vi "Load Class From Config.vi"(8 "error in (no error)":errorcluster, 11 "Name":string) -> (0 "error out":errorcluster, 2 "Success":bool, 3 "Channel":refnum<class "Channel.lvclass">)   [LabVIEW 2021, in "Channel.lvlib"]
doc: "Loads the class from the configuration Folder"
uses:
  Channel.lvlib
  Channel/Channel_class/Channel.lvclass
  <vilib>/Utility/config.llb/Read Key (String).vi
  <vilib>/Utility/config.llb/NI_LVConfig.lvlib
panel:
  in  "PluginPath(T)":bool=TRUE
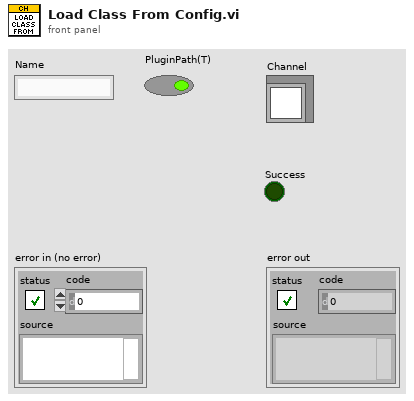
[diagram p1: front panel]
types:
  T1 = typedef "NI_LVConfig.lvlib/Config Data RefNum.ctl" = refnum<k1>
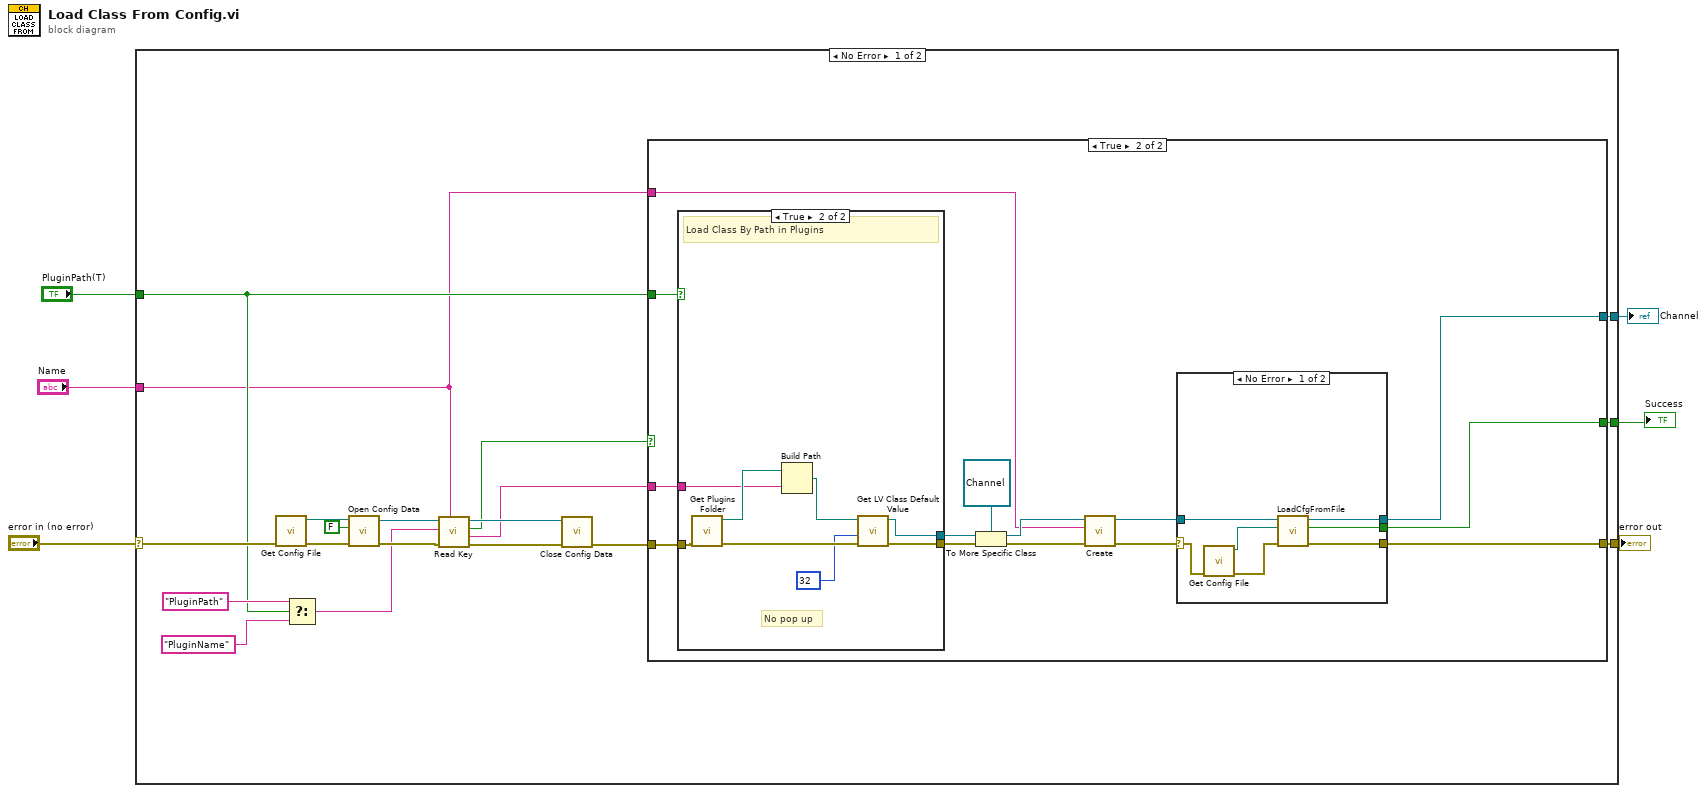
[diagram p0: block diagram]
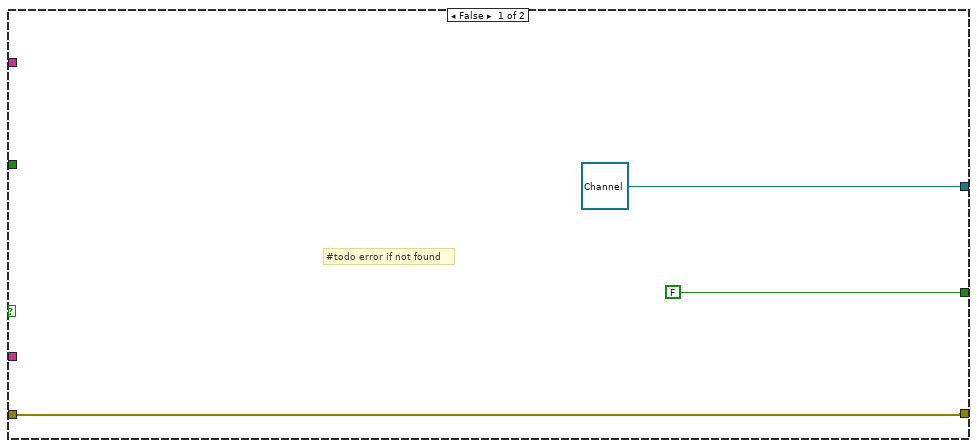
[diagram p2: hidden frame]
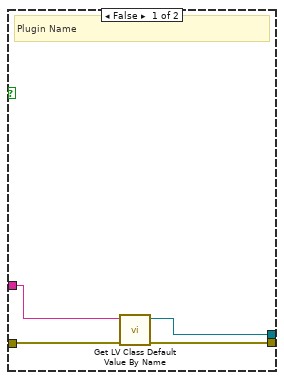
[diagram p3: hidden frame]
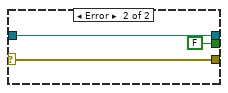
[diagram p4: hidden frame]
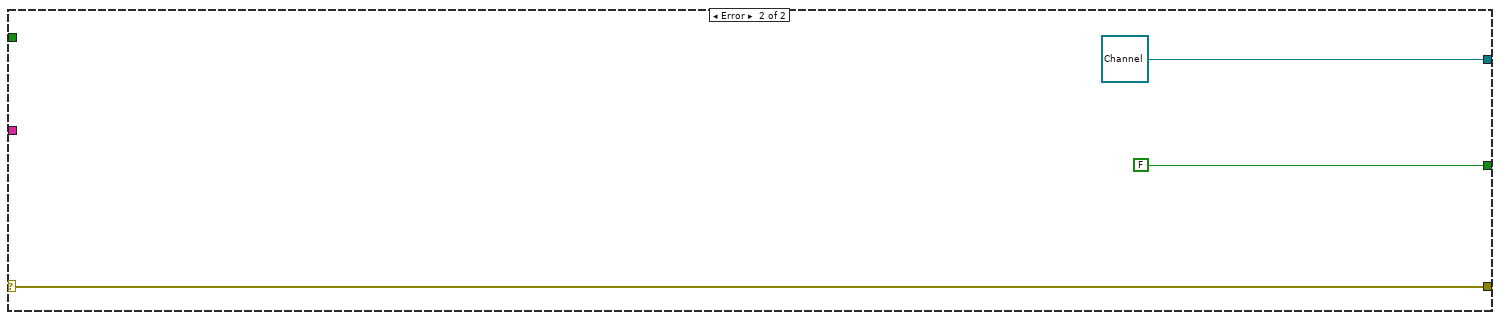
[diagram p5: hidden frame]
diagram:
  n1 = case shown="No Error" "error in (no error)" {
    selector: "error in (no error)" -> [w25 w66]
    tunnel: [w24 w66] -> w5
    tunnel: "Name" -> [w7 _]
    tunnel: [w12 FALSE ("Boolean")] -> w3
    tunnel: [w11 refnum<class "Channel.lvclass"> refnum ("Channel.lvlib:Channel")] -> w2
    tunnel: "PluginPath(T)" -> [w9 _]
    frame No Error {
      n2 = call "Get Config File.vi"("error in (no error)"=w25) -> ("error out"=w18:errorcluster, "Config File"=w21:path)  [unwired: 9 in]
      n3 = Select(t="PluginPath" ("key"), s=w9, f="PluginName") -> (s? t:f=w10:string)
      n4 = call <vilib>:"Open Config Data.vi"("error in (no error)"=w18, "create file if necessary (T)"=FALSE, "configuration file path"=w21) -> ("error out"=w19:errorcluster, "refnum"=w22:T1)  [unwired: 6 in, 1 out]
      n5 = call-poly <vilib>:"Read Key.vi"("section"=w7, "error in (no error)"=w19, "key"=w10, "refnum"=w22) -> ("error out"=w16:errorcluster, "value"=w14:string, "found?"=w13:bool, "refnum out"=w23:T1)  [unwired: 4 in]
      n6 = call <vilib>:"Close Config Data.vi"("error in (no error)"=w16, "refnum"=w23) -> ("error out"=w17:errorcluster)  [unwired: 8 in, 1 out]
      n7 = case shown="True" w13 {
        tunnel: [w28 w36] -> w24
        tunnel: w17 -> [w28 w42]
        tunnel: w14 -> [_ w41]
        tunnel: [FALSE ("Boolean") w35] -> w12
        tunnel: [refnum<class "Channel.lvclass"> refnum ("Channel.lvlib:Channel") w37] -> w11
        tunnel: w9 -> [_ w34]
        tunnel: w7 -> [_ w29]
        frame False {
          # "#todo error if not found"
        }
        frame True {
          n8 = case shown="True" w34 {
            tunnel: w42 -> [w45 w54]
            tunnel: w41 -> [w46 w52]
            tunnel: [w43 w49] -> w39
            tunnel: [w44 w48] -> w38
            frame False {
              # "Plugin Name"
              n9 = call <vilib>:"Get LV Class Default Value By Name.vi"("error in (no error)"=w45, "class name"=w46) -> ("error out"=w44:errorcluster, "object"=w43:refnum<class>)  [unwired: 8 in]
            }
            frame True {
              # "No pop up"
              # "Load Class By Path in Plugins"
              n10 = call "Get Plugins Folder.vi"("error in (no error)"=w54) -> ("error out"=w50:errorcluster, "Plugins Folder"=w53:path)  [unwired: 9 in]
              n11 = Build Path(base path=w53, name or relative path=w52) -> (appended path=w51:path)
              n12 = call <vilib>:"Get LV Class Default Value.vi"("error in (no error)"=w50, "options"=u32 32, "class path"=w51) -> ("error out"=w48:errorcluster, "object"=w49:refnum<class>)  [unwired: 7 in]
            }
          }
          n13 = To More Specific Class(target class=refnum<class "Channel.lvclass"> refnum ("Channel.lvlib:Channel"), reference=w39, error in=w38) -> (specific class reference=w33:refnum<class "Channel.lvclass">, error out=w32:errorcluster)
          n14 = call-dynamic "Create.vi"("error in (no error)"=w32, "Name"=w29, "object in"=w33) -> ("error out"=w31:errorcluster, "object out"=w30:refnum<class "Channel.lvclass">)  [unwired: 7 in]
          n15 = case shown="No Error" w31 {
            selector: w31 -> [w58 w63]
            tunnel: w30 -> [w61 w64]
            tunnel: [w60 w64] -> w37
            tunnel: [w59 w63] -> w36
            tunnel: [w55 FALSE ("Success?")] -> w35
            frame No Error {
              n16 = call "Get Config File.vi"("error in (no error)"=w58) -> ("error out"=w57:errorcluster, "Config File"=w56:path)  [unwired: 9 in]
              n17 = call-dynamic "LoadCfgFromFile.vi"("error in (no error)"=w57, "Configuration FIle"=w56, "object in"=w61) -> ("error out"=w59:errorcluster, "Success?"=w55:bool, "object out"=w60:refnum<class "Channel.lvclass">)  [unwired: 6 in]
            }
            frame Error {
            }
          }
        }
      }
    }
    frame Error {
    }
  }
  "error out" <- w5
  "Success" <- w3
  "Channel" <- w2
